vi "RT_lab9.vi"() -> ()   [LabVIEW 2025]
uses:
  states.ctl
panel:
  out "Disk  [%]":dbl
  out "CPU [%]":dbl
  out "Elements Remaining":u32
  out "Waveform Graph":i16[][](graph)
  out "error out":errorcluster
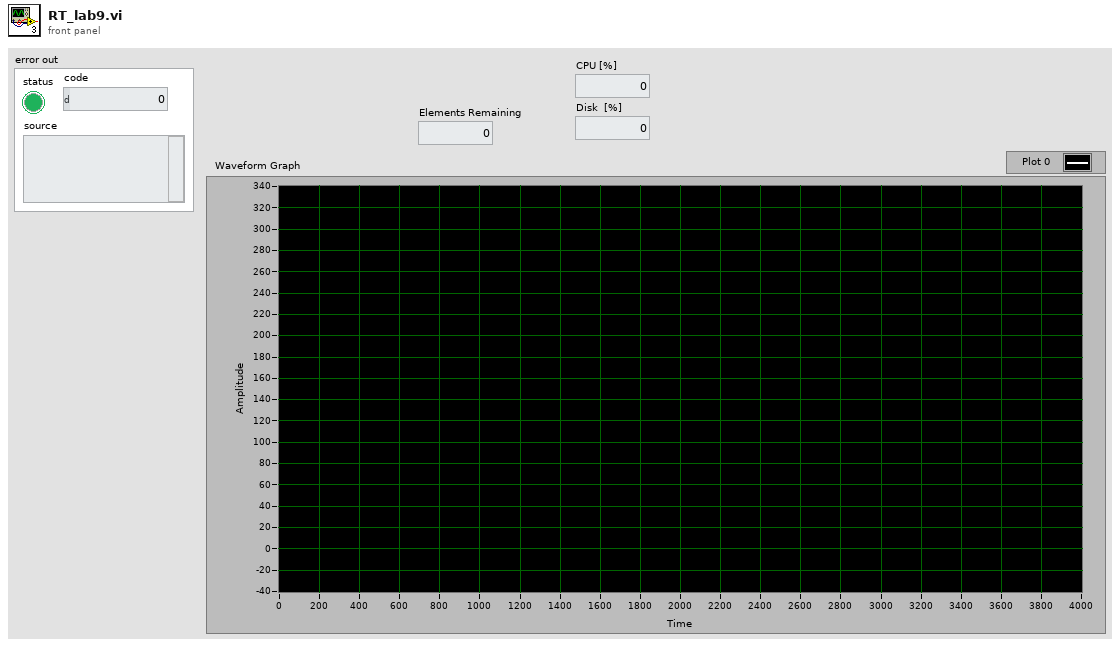
[diagram p1: front panel]
types:
  T1 = typedef "states.ctl" = enum16{"Run", "Connect"}
  T2 = typedef "Logger_State.ctl" = cluster{"ref TDMS":refnum<k34>, "File Path":path, "counter":i32, "Folder tmp":path, "folder ready":path}
  T3 = typedef "RT_Cmd.ctl" = cluster{"command":T4, "parameters":T5, "file name":string}
  T4 = typedef "Command.ctl" = enum16{"threshold_config", "manual_trigger", "stop", "remove_file"}
  T5 = typedef "thresholds.ctl" = cluster{"Thr_X":i16, "Thr_Y":i16, "Thr_Z":i16}
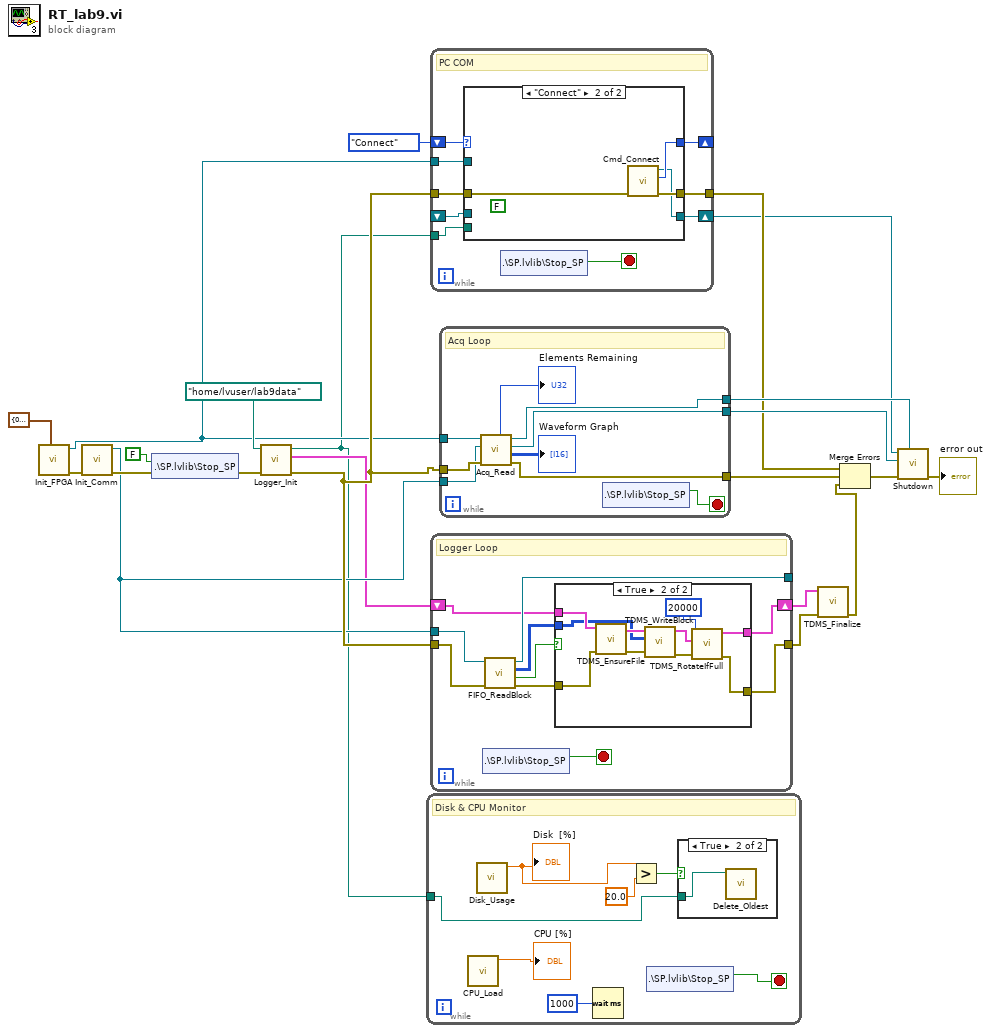
[diagram p0: block diagram]
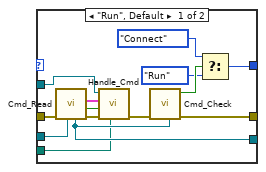
[diagram p3: hidden frame]
diagram:
  n1 = call "Init_FPGA.vi"("Threshold"=cluster{"Thr_X":i16, "Thr_Y":i16, "Thr_Z":i16} {"Thr_X"=0, "Thr_Y"=0, "Thr_Z"=0}) -> ("error out"=w21:errorcluster, "FPGA VI Reference Out"=w7:refnum<k20>)  [unwired: 9 in]
  n2 = call "Init_Comm.vi"("error in"=w21) -> ("error out"=w17:errorcluster, "rt fifo ref out"=w6:refnum<k33>)  [unwired: 9 in]
  n3 = shared-variable ".\\SP.lvlib\\Stop_SP"(FALSE ("Stop_SP"), error in=w17) -> (error out=w10:errorcluster)
  n4 = call "Logger_Init.vi"("error in (no error)"=w10, "base path"=path "/home/lvuser/lab9data") -> ("error out"=w9:errorcluster, "state"=w5:T2, "Folder ready"=w4:path)  [unwired: 7 in]
  n5 = while {
    tunnel: w4 -> [w24]
    stop <- w29 stop-if-true
    # "Disk & CPU Monitor"
    n6 = call "CPU_Load.vi"() -> ("CPU [%]"=→"CPU [%]":dbl)  [unwired: 11 in]
    n7 = call "Disk_Usage.vi"() -> ("usage %"=w27:dbl)  [unwired: 11 in]
    "Disk  [%]" <- w27
    n8 = Wait (ms)(milliseconds to wait=u32 1000) -> ()  [unwired: 1 out]
    n9 = Greater?(x=w27, y=20.0) -> (0:w25:bool)
    n10 = shared-variable ".\\SP.lvlib\\Stop_SP"() -> (w29:bool)  [unwired: 1 in, 1 out]
    n11 = case shown="True" w25 {
      tunnel: w24 -> [_ w30]
      frame False {
      }
      frame True {
        n12 = call "Delete_Oldest.vi"("Folder ready"=w30) -> ()  [unwired: 11 in]
      }
    }
  }
  n13 = while {
    tunnel: w9 -> [w38]
    tunnel: w7 -> [w37]
    shift-right: [w36] -> _
    shift-left: states."Connect" -> [w39]
    tunnel: [w35] -> w12
    shift-right: [w34] -> w11
    shift-left: _ -> [w33]
    tunnel: w4 -> [w31]
    stop <- w32 stop-if-true
    # "PC COM"
    n14 = case shown="\"Connect\"" w39 {
      tunnel: w38 -> [w53 w57]
      tunnel: w37 -> [w40 _]
      tunnel: [w52 w56] -> w35
      tunnel: [w42 w55] -> w36
      tunnel: [w46 w54] -> w34
      tunnel: w33 -> [w47 _]
      tunnel: w31 -> [w41 _]
      frame "Run", Default {
        n15 = call "Cmd_Read.vi"("Refnum in"=w47, "error in (no error)"=w53) -> ("error out"=w49:errorcluster, "timed out?"=w50:bool, "data out"=w51:T3, "Refnum out"=w46:refnum<k21>)  [unwired: 6 in]
        n16 = call "Handle_Cmd.vi"("folder ready"=w41, "error in"=w49, "timed out?"=w50, "data IN"=w51, "FPGA VI Reference IN"=w40) -> ("error out"=w48:errorcluster)  [unwired: 5 in, 1 out]
        n17 = call "Cmd_Check.vi"("Refnum in"=w46, "error in (no error)"=w48) -> ("error out"=w52:errorcluster, "disconnected?"=w45:bool)  [unwired: 8 in]
        n18 = Select(t=states."Connect", s=w45, f=states."Run") -> (s? t:f=w42:T1)
      }
      frame "Connect" {
        (unwired) FALSE
        n19 = call "Cmd_Connect.vi"("error in (no error)"=w57) -> ("error out"=w56:errorcluster, "Enum"=w55:T1, "Refnum out"=w54:refnum<k21>)  [unwired: 8 in]
      }
    }
    n20 = shared-variable ".\\SP.lvlib\\Stop_SP"() -> (w32:bool)  [unwired: 1 in, 1 out]
  }
  n21 = while {
    tunnel: w9 -> [w65]
    tunnel: [w59] -> w3
    tunnel: w6 -> [w66]
    shift-right: [w58] -> w1
    shift-left: w5 -> [w61]
    tunnel: [w62] -> _
    stop <- w67 stop-if-true
    # "Logger Loop"
    n22 = shared-variable ".\\SP.lvlib\\Stop_SP"() -> (w67:bool)  [unwired: 1 in, 1 out]
    n23 = call "FIFO_ReadBlock.vi"("error in (no error)"=w65, "rt fifo ref in"=w66) -> ("error out"=w60:errorcluster, "blok?"=w64:bool, "dane"=w63:i16[][], "rt fifo ref out"=w62:refnum<k33>)  [unwired: 6 in]
    n24 = case shown="True" w64 {
      tunnel: w63 -> [_ w75]
      tunnel: w61 -> [w68 w79]
      tunnel: w60 -> [w69 w78]
      tunnel: [w69 w71] -> w59
      tunnel: [w68 w70] -> w58
      frame False {
      }
      frame True {
        n25 = call "TDMS_EnsureFile.vi"("error in (no error)"=w78, "Logger_state"=w79) -> ("error out"=w77:errorcluster, "state out"=w76:T2)  [unwired: 8 in]
        n26 = call "TDMS_WriteBlock.vi"("error in (no error)"=w77, "Array"=w75, "Logger_state"=w76) -> ("error out"=w74:errorcluster, "state out"=w73:T2)  [unwired: 7 in]
        n27 = call "TDMS_RotateIfFull.vi"("error in (no error)"=w74, "state in"=w73, "max samples"=20000) -> ("error out"=w71:errorcluster, "state out"=w70:T2)  [unwired: 7 in]
      }
    }
  }
  n28 = while {
    tunnel: w7 -> [w88]
    tunnel: w9 -> [w87]
    tunnel: [w86] -> w19
    tunnel: [w84] -> w13
    tunnel: w6 -> [w85]
    tunnel: [w83] -> w18
    stop <- w82 stop-if-true
    # "Acq Loop"
    n29 = call "Acq_Read.vi"("error in (no error)"=w87, "rt fifo ref in"=w85, "Refnum in"=w88) -> ("error out"=w84:errorcluster, "Array"=→"Waveform Graph":i16[][], "rt fifo ref out"=w83:refnum<k33>, "FPGA VI Reference Out"=w86:refnum<k20>, "Elements Remaining"=→"Elements Remaining":u32)  [unwired: 4 in]
    n30 = shared-variable ".\\SP.lvlib\\Stop_SP"() -> (w82:bool)  [unwired: 1 in, 1 out]
  }
  n31 = call "TDMS_Finalize.vi"("error in (no error)"=w3, "state in"=w1) -> ("error out"=w2:errorcluster)  [unwired: 9 in]
  n32 = Merge Errors(w12, w13, w2) -> (w20:errorcluster)
  n33 = call "Shutdown.vi"("FPGA ref"=w19, "error in (no error)"=w20, "rt fifo ref in"=w18, "cdm reader"=w11) -> ("error out"=→"error out":errorcluster)  [unwired: 7 in]
